vi "Load Config.vi"(8 "error in (no error)":errorcluster, 11 "Sift TDMS Uploader in":refnum<class "Sift TDMS Uploader.lvclass">) -> (0 "error out":errorcluster, 3 "Sift TDMS Uploader out":refnum<class "Sift TDMS Uploader.lvclass">)   [LabVIEW 2024, in "Sift TDMS Uploader.lvlib" / "Sift TDMS Uploader.lvclass"]
uses:
  Sift TDMS Uploader.lvclass
  <vilib>/Utility/sysdir.llb/System Directory Type.ctl
  Sift TDMS Uploader.lvclass/Sift TDMS Uploader.ctl
  <vilib>/Utility/config.llb/Read Key (String).vi
  <vilib>/Utility/config.llb/NI_LVConfig.lvlib
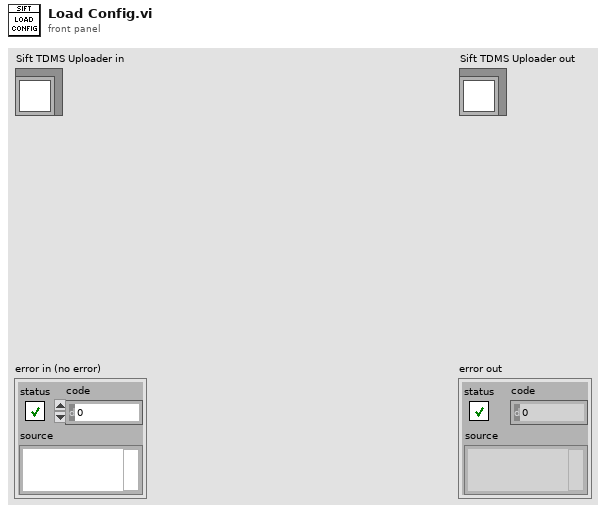
[diagram p1: front panel]
types:
  T1 = typedef "System Directory Type.ctl" = i32
  T2 = typedef "NI_LVConfig.lvlib/Config Data RefNum.ctl" = refnum<k1>
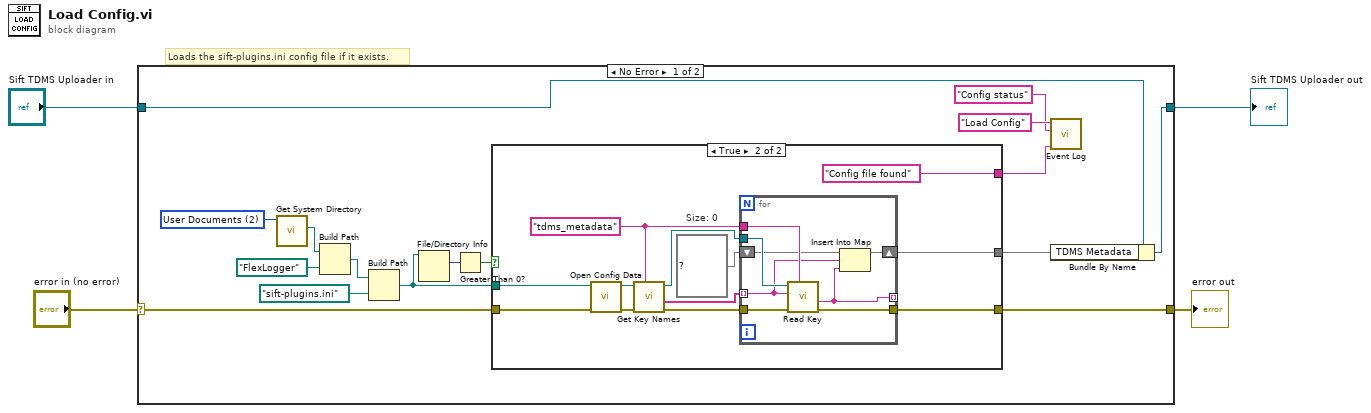
[diagram p0: block diagram]
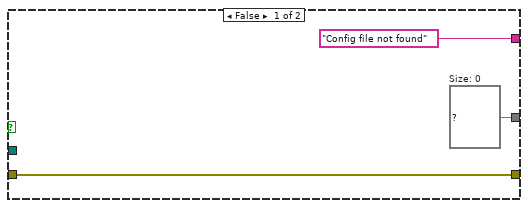
[diagram p2: hidden frame]
diagram:
  # "Loads the sift-plugins.ini config file if it exists."
  n1 = case shown="No Error" "error in (no error)" {
    selector: "error in (no error)" -> [w12 w45]
    tunnel: [w8 w45] -> w3
    tunnel: [w9 w44] -> w1
    tunnel: "Sift TDMS Uploader in" -> [w11 w44]
    frame No Error {
      w20 = T1 2 items=["User Home"=0, "User Desktop"=1, "User Documents"=2, "User Application Data"=3, "User Preferences"=4, "User Temporary"=5, "Public Documents"=6, "Public Application Data"=7, "Public Preferences"=8, "Public Cache"=13, "System Core Libraries"=9, "System Installed Libraries"=10, "Application Files"=11, "Boot Volume Root"=12] ("system directory type")
      n2 = call <vilib>:"Get System Directory.vi"("system directory type"=w20) -> ("system directory"=w19:path)  [unwired: 10 in]
      n3 = Build Path(base path=w19, name or relative path=path "FlexLogger") -> (appended path=w17:path)
      n4 = Build Path(base path=w17, name or relative path=path "sift-plugins.ini") -> (appended path=w13:path)
      n5 = File/Directory Info(path=w13) -> (size=w15:i64)  [unwired: 1 in, 6 out]
      n6 = Greater Than 0?(x=w15) -> (x > 0?=w14:bool)
      n7 = case shown="True" w14 {
        tunnel: w13 -> [_ w28]
        tunnel: w12 -> [w22 w27]
        tunnel: [w23 w26] -> w10
        tunnel: [w22 w25] -> w8
        tunnel: ["Config file not found" "Config file found"] -> w5
        frame False {
          w23 = map{string, string} {}  # Size: 0
        }
        frame True {
          w29 = map{string, string} {}  # Size: 0
          w30 = "tdms_metadata" ("section")
          n8 = call <vilib>:"Open Config Data.vi"("error in (no error)"=w27, "configuration file path"=w28) -> ("error out"=w32:errorcluster, "refnum"=w31:T2)  [unwired: 7 in, 1 out]
          n9 = call <vilib>:"Get Key Names.vi"("section"=w30, "error in (no error)"=w32, "refnum"=w31) -> ("error out"=w35:errorcluster, "key names"=w33:string[], "refnum out"=w34:T2)  [unwired: 5 in, 1 out]
          n10 = for {
            tunnel: w33 -> [w39] mode=indexing
            tunnel: w34 -> [w43]
            tunnel: w30 -> [w42]
            tunnel: w35 -> [w41]
            tunnel: [w40] -> w25
            tunnel: [w38] -> _ mode=indexing
            shift-right: [w37] -> w26
            shift-left: w29 -> [w36]
            n11 = call-poly <vilib>:"Read Key.vi"("section"=w42, "error in (no error)"=w41, "key"=w39, "refnum"=w43) -> ("error out"=w40:errorcluster, "value"=w38:string)  [unwired: 4 in, 2 out]
            n12 = Insert Into Map(map in=w36, key=w39, value=w38) -> (map out=w37:map{string, string})  [unwired: 2 out]
          }
        }
      }
      n13 = call "Event Log.vi"("Message"=w5, "Event Type"="Config status", "Location"="Load Config") -> ()  [unwired: 9 in]
      n14 = Bundle By Name(cluster=w11, "TDMS Metadata"=w10) -> (w9:refnum<class "Sift TDMS Uploader.lvclass">)
    }
    frame Error {
    }
  }
  "error out" <- w3
  "Sift TDMS Uploader out" <- w1
